vi "SMTP Email [VRFY].vi"(4 "error in (no error)":errorcluster caption="entrée d'erreur (pas d'erreur)", 6 "user":string caption="utilisateur", 7 "smtp session":T1 caption="session smtp") -> (0 "error out":errorcluster caption="sortie d'erreur", 1 "reply":string caption="réponse", 2 "reply code":i32 caption="code de réponse", 3 "smtp session out":T1 caption="session smtp en sortie")   [LabVIEW 2022 SP3, in "Copie de NI_SMTPEmail.lvlib"]
doc: "Envoie la commande VRFY au serveur SMTP via connexion TCP décrite par \"ID de connexion\", reçoit la réponse et l'interprète.\n\nCe VI renvoie \"ID de connexion en sortie\" et les résultats d'interprétation de l'erreur dans le cluster de \"sortie d'erreur\"."
uses:
  Copie de NI_SMTPEmail.lvlib
  SMTP Email Session.ctl
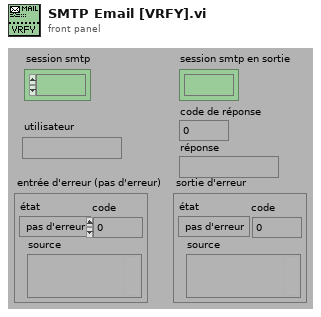
[diagram p1: front panel]
types:
  T1 = typedef "Copie de NI_SMTPEmail.lvlib/SMTP Email Session.ctl" = refnum<k1>
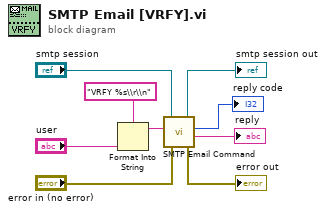
[diagram p0: block diagram]
diagram:
  n1 = Format Into String(format string="VRFY %s\\r\\n", "user") -> (resulting string=w2:string)  [unwired: 2 in, 1 out]
  n2 = call "SMTP Email Command.vi"("error in (no error)"="error in (no error)", "command"=w2, "smtp session"="smtp session") -> ("error out"=→"error out":errorcluster, "reply"=→"reply":string, "reply code"=→"reply code":i32, "smtp session out"=→"smtp session out":T1)  [unwired: 1 in]
